vi "query Measurement Trace Values into CSV File.vi"(8 "error in (no error)":errorcluster, 9 "Trace Index":i32, 10 "Path":path, 11 "Keysight 9020A in":refnum<class "Keysight 9020A.lvclass">) -> (0 "error out":errorcluster, 3 "Keysight 9020A out":refnum<class "Keysight 9020A.lvclass">)   [LabVIEW 2023, in "Spectrum Analyzer.lvlib" / "Keysight 9020A.lvclass"]
uses:
  Keysight 9020A.lvclass
  Keysight 9020A.lvclass/Keysight 9020A.ctl
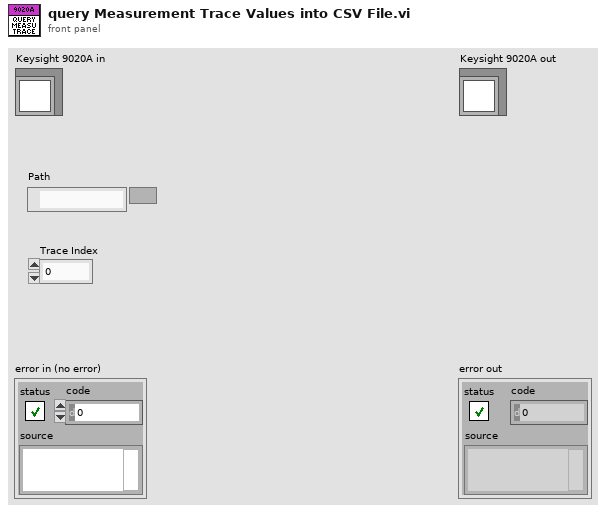
[diagram p1: front panel]
types:
  T1 = enum16{"big-endian, network order", "native, host order", "little-endian"}
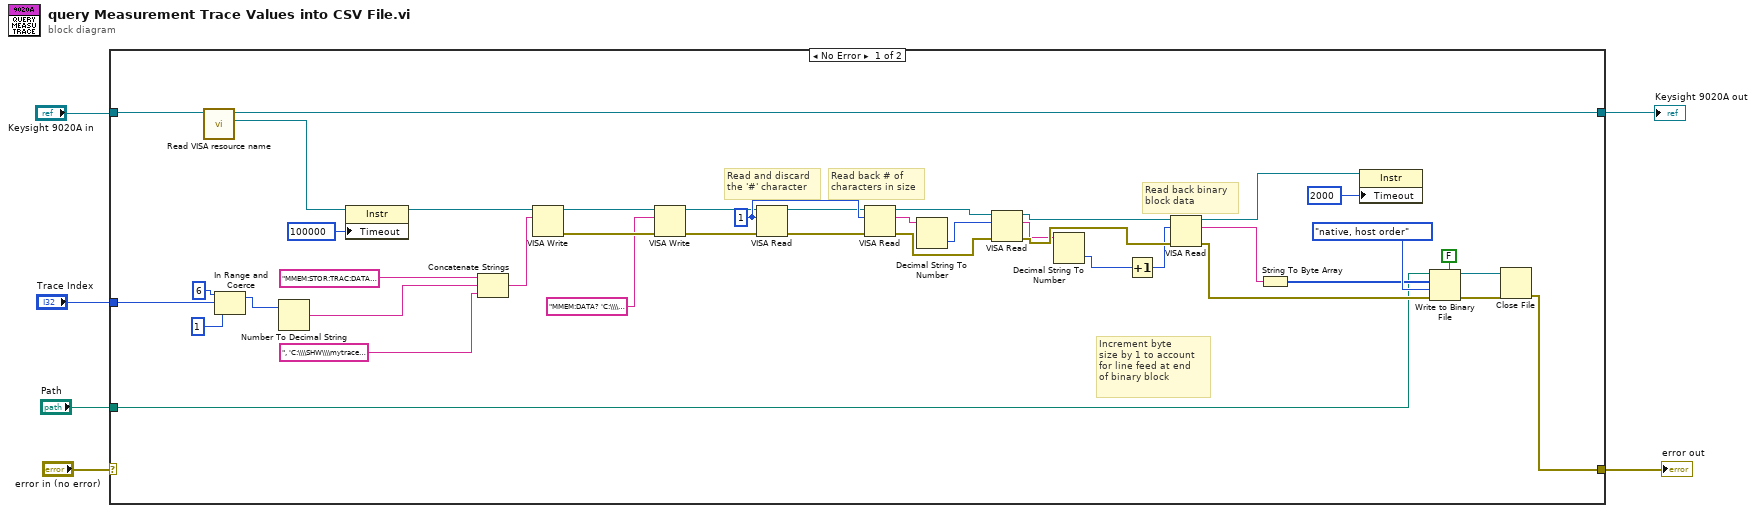
[diagram p0: block diagram]
diagram:
  n1 = case shown="No Error" "error in (no error)" {
    selector: "error in (no error)" -> [_ w48]
    tunnel: "Keysight 9020A in" -> [w46 w49]
    tunnel: [w47 w49] -> w5
    tunnel: [w9 w48] -> w3
    tunnel: "Trace Index" -> [w36 _]
    tunnel: "Path" -> [w7 _]
    frame No Error {
      w19 = u32 1 ("byte count")
      # "Read back binary\nblock data"
      # "Increment byte\nsize by 1 to account\nfor line feed at end\nof binary block"
      # "Read back # of\ncharacters in size"
      # "Read and discard\nthe '#' character"
      n2 = call "Read VISA resource name.vi"("Keysight 9020A in"=w46) -> ("VISA resource name"=w44:refnum<visa-resource-name>, "Keysight 9020A out"=w47:refnum<class "Keysight 9020A.lvclass">)  [unwired: 8 in, 1 out]
      n3 = In Range and Coerce(upper limit=6, x=w36, lower limit=1) -> (coerced(x)=w37:i32)  [unwired: 1 out]
      n4 = Number To Decimal String(number=w37) -> (decimal integer string=w41:string)  [unwired: 1 in]
      n5 = property class="Instr"(reference=w44, "Timeout"=u32 100000 ("General Settings:Timeout Value")) -> (reference out=w43:refnum<visa-resource-name>)  [unwired: 1 in, 1 out]
      n6 = Concatenate Strings("MMEM:STOR:TRAC:DATA TRACE" ("write buffer"), w41, ", 'C:\\\\SHW\\\\mytrace.csv';*OPC" ("write buffer")) -> (w35:string)
      n7 = VISA Write(VISA resource name=w43, write buffer=w35) -> (VISA resource name out=w13:refnum<visa-resource-name>, error out=w12:errorcluster)  [unwired: 1 in, 1 out]
      n8 = VISA Write(VISA resource name=w13, write buffer="MMEM:DATA? 'C:\\\\SHW\\\\mytrace.csv'", error in (no error)=w12) -> (VISA resource name out=w16:refnum<visa-resource-name>, error out=w15:errorcluster)  [unwired: 1 out]
      n9 = VISA Read(VISA resource name=w16, byte count=w19, error in (no error)=w15) -> (VISA resource name out=w17:refnum<visa-resource-name>, error out=w18:errorcluster)  [unwired: 2 out]
      n10 = VISA Read(VISA resource name=w17, byte count=w19, error in (no error)=w18) -> (VISA resource name out=w29:refnum<visa-resource-name>, read buffer=w20:string, error out=w30:errorcluster)  [unwired: 1 out]
      n11 = Decimal String To Number(string=w20) -> (number=w28:i32)  [unwired: 2 in, 1 out]
      n12 = VISA Read(VISA resource name=w29, byte count=w28, error in (no error)=w30) -> (VISA resource name out=w31:refnum<visa-resource-name>, read buffer=w32:string, error out=w34:errorcluster)  [unwired: 1 out]
      n13 = Decimal String To Number(string=w32) -> (number=w33:i32)  [unwired: 2 in, 1 out]
      n14 = Increment(x=w33) -> (x+1=w21:i32)
      n15 = VISA Read(VISA resource name=w31, byte count=w21, error in (no error)=w34) -> (VISA resource name out=w11:refnum<visa-resource-name>, read buffer=w25:string, error out=w10:errorcluster)  [unwired: 1 out]
      n16 = String To Byte Array(string=w25) -> (unsigned byte array=w26:u8[])
      n17 = property class="Instr"(reference=w11, "Timeout"=u32 2000 ("General Settings:Timeout Value")) -> ()  [unwired: 1 in, 2 out]
      n18 = Write to Binary File(file (use dialog)=w7, data=w26, error in=w10, 5:FALSE ("prepend array or string size? (T)"), 9:T1."native, host order" ("byte order (0:big-endian, network order)")) -> (refnum out=w24:refnum<file>, error out=w23:errorcluster)  [unwired: 1 in, 1 out]
      n19 = Close File(refnum=w24, error in=w23) -> (error out=w9:errorcluster)  [unwired: 1 out]
    }
    frame Error {
    }
  }
  "error out" <- w3
  "Keysight 9020A out" <- w5
